vi "run.vi"(8 "error in (no error)":errorcluster, 11 "Filter_Wheel in":refnum<class "Filter_Wheel.lvclass">) -> (0 "error out":errorcluster, 3 "Filter_Wheel out":refnum<class "Filter_Wheel.lvclass">)   [LabVIEW 2018, in "Filter_Wheel.lvclass"]
uses:
  Filter_Wheel.lvclass
  Filter_Wheel.lvclass/Filter_Wheel.ctl
  State Machine/State Machine.lvclass/State Machine.ctl
  State Machine/State Machine.lvclass
  RxTx/RxTx.lvclass
panel:
  out "Select Filter":u16(ring) items=["Methane", "U", "B", "V", "R", "I", "Clear"]
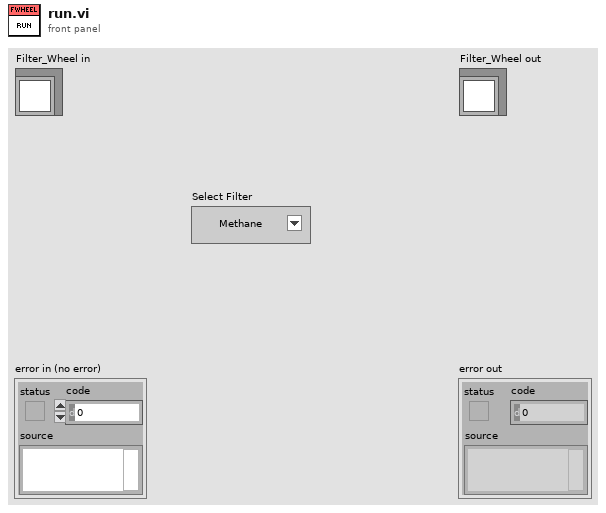
[diagram p1: front panel]
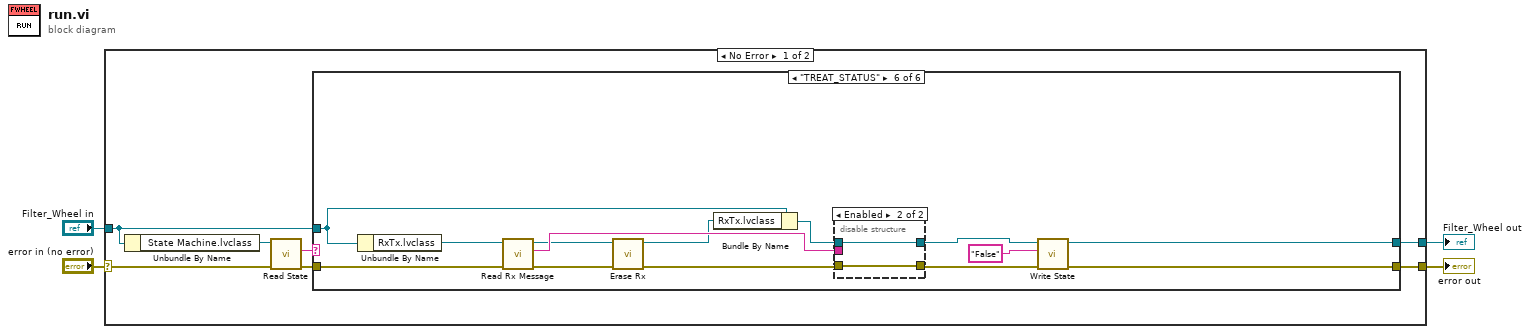
[diagram p0: block diagram]
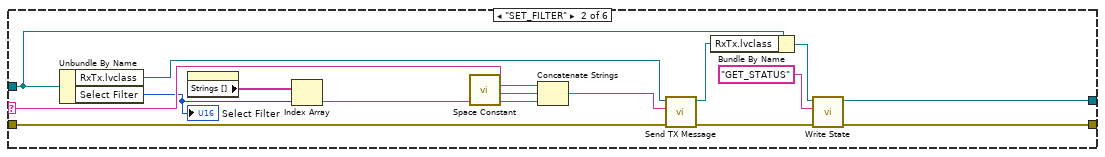
[diagram p3: hidden frame]
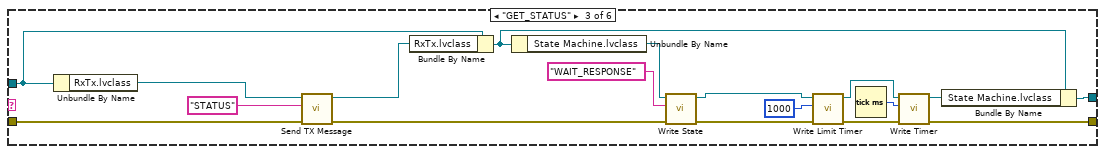
[diagram p4: hidden frame]
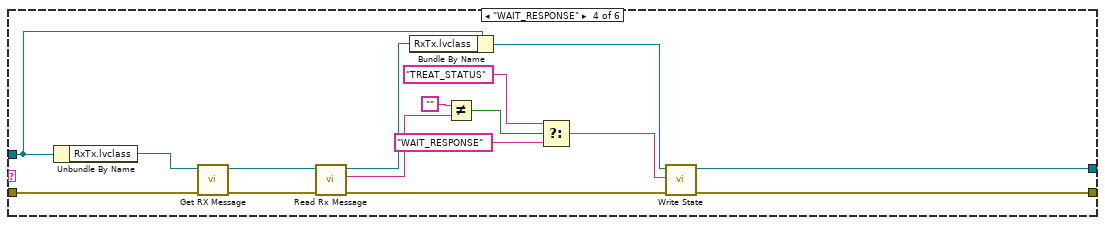
[diagram p5: hidden frame]
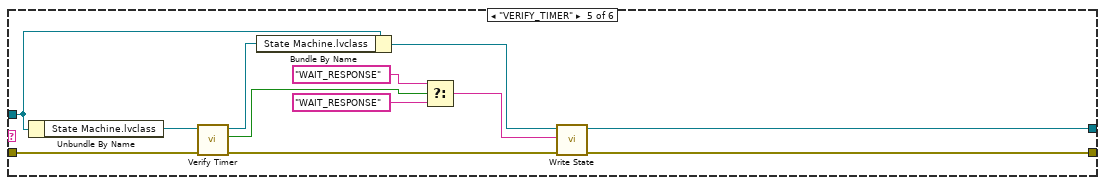
[diagram p6: hidden frame]
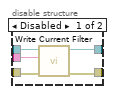
[diagram p7: hidden frame]
diagram:
  n1 = case shown="No Error" "error in (no error)" {
    selector: "error in (no error)" -> [w10 w97]
    tunnel: [w5 w97] -> w3
    tunnel: [w6 w96] -> w1
    tunnel: "Filter_Wheel in" -> [w8 w96]
    frame No Error {
      n2 = Unbundle By Name(w8) -> ("State Machine.lvclass"=w11:refnum<class "State Machine.lvclass">)
      n3 = call-dynamic "Read State.vi"("error in (no error)"=w10, "State Machine in"=w11) -> ("error out"=w7:errorcluster, "State"=w9:string)  [unwired: 7 in, 1 out]
      n4 = case shown="\"TREAT_STATUS\"" w9 {
        selector: w9 -> [_ w27 _ _ _ _]
        tunnel: w8 -> [w13 w24 w42 w62 w74 w88]
        tunnel: w7 -> [w12 w25 w46 w57 w66 w84]
        tunnel: [w13 w18 w37 w59 w71 w86] -> w6
        tunnel: [w12 w19 w38 w60 w72 w87] -> w5
        frame "False", Default {
        }
        frame "SET_FILTER" {
          n5 = Unbundle By Name(w24) -> ("RxTx.lvclass"=w22:refnum<class "RxTx.lvclass">, "Select Filter"=w15:u16)
          "Select Filter" <- w15
          n6 = property on="Select Filter" class="Ring (strict)"() -> ("Strings []"=w16:string[])  [unwired: 2 in, 2 out]
          n7 = Index Array(array=w16, index=w15) -> (element=w14:string)
          n8 = call <vilib>:"Space Constant.vi"() -> ("String"=w26:string)
          n9 = Concatenate Strings(w27, w26, w14) -> (w28:string)
          n10 = call "Send TX Message.vi"("error in (no error)"=w25, "element"=w28, "RxTx in"=w22) -> ("error out"=w20:errorcluster, "RxTx out"=w23:refnum<class "RxTx.lvclass">)  [unwired: 7 in]
          n11 = Bundle By Name(cluster=w24, "RxTx.lvclass"=w23) -> (w21:refnum<class "Filter_Wheel.lvclass">)
          n12 = call "Write State.vi"("error in (no error)"=w20, "State"="GET_STATUS", "Filter_Wheel in"=w21) -> ("error out"=w19:errorcluster, "Filter_Wheel out"=w18:refnum<class "Filter_Wheel.lvclass">)  [unwired: 7 in]
        }
        frame "GET_STATUS" {
          n13 = Unbundle By Name(w42) -> ("RxTx.lvclass"=w44:refnum<class "RxTx.lvclass">)
          n14 = call "Send TX Message.vi"("error in (no error)"=w46, "element"="STATUS", "RxTx in"=w44) -> ("error out"=w41:errorcluster, "RxTx out"=w45:refnum<class "RxTx.lvclass">)  [unwired: 7 in]
          n15 = Bundle By Name(cluster=w42, "RxTx.lvclass"=w45) -> (w32:refnum<class "Filter_Wheel.lvclass">)
          n16 = Unbundle By Name(w32) -> ("State Machine.lvclass"=w33:refnum<class "State Machine.lvclass">)
          n17 = call-dynamic "Write State.vi"("error in (no error)"=w41, "State"="WAIT_RESPONSE", "State Machine in"=w33) -> ("error out"=w40:errorcluster, "State Machine out"=w34:refnum<class "State Machine.lvclass">)  [unwired: 7 in]
          n18 = call "Write Limit Timer.vi"("error in (no error)"=w40, "Limit Timer"=u32 1000, "State Machine in"=w34) -> ("error out"=w39:errorcluster, "State Machine out"=w35:refnum<class "State Machine.lvclass">)  [unwired: 7 in]
          n19 = Tick Count (ms)() -> (millisecond timer value=w29:u32)
          n20 = call "Write Timer.vi"("error in (no error)"=w39, "Timer"=w29, "State Machine in"=w35) -> ("error out"=w38:errorcluster, "State Machine out"=w36:refnum<class "State Machine.lvclass">)  [unwired: 7 in]
          n21 = Bundle By Name(cluster=w32, "State Machine.lvclass"=w36) -> (w37:refnum<class "Filter_Wheel.lvclass">)
        }
        frame "WAIT_RESPONSE" {
          n22 = Unbundle By Name(w62) -> ("RxTx.lvclass"=w58:refnum<class "RxTx.lvclass">)
          n23 = call "Get RX Message.vi"("error in (no error)"=w57, "RxTx in"=w58) -> ("error out"=w56:errorcluster, "RxTx out"=w55:refnum<class "RxTx.lvclass">)  [unwired: 8 in]
          n24 = call "Read Rx Message.vi"("error in (no error)"=w56, "RxTx in"=w55) -> ("error out"=w48:errorcluster, "Rx Message"=w54:string, "RxTx out"=w47:refnum<class "RxTx.lvclass">)  [unwired: 7 in]
          n25 = Bundle By Name(cluster=w62, "RxTx.lvclass"=w47) -> (w61:refnum<class "Filter_Wheel.lvclass">)
          n26 = Not Equal?(x="", y=w54) -> (x != y?=w52:bool)
          n27 = Select(t="TREAT_STATUS" ("State"), s=w52, f="WAIT_RESPONSE" ("State")) -> (s? t:f=w49:string)
          n28 = call "Write State.vi"("error in (no error)"=w48, "State"=w49, "Filter_Wheel in"=w61) -> ("error out"=w60:errorcluster, "Filter_Wheel out"=w59:refnum<class "Filter_Wheel.lvclass">)  [unwired: 7 in]
        }
        frame "VERIFY_TIMER" {
          n29 = Unbundle By Name(w74) -> ("State Machine.lvclass"=w67:refnum<class "State Machine.lvclass">)
          n30 = call "Verify Timer.vi"("error in (no error)"=w66, "State Machine in"=w67) -> ("error out"=w65:errorcluster, "time out"=w63:bool, "State Machine out"=w64:refnum<class "State Machine.lvclass">)  [unwired: 7 in]
          n31 = Bundle By Name(cluster=w74, "State Machine.lvclass"=w64) -> (w73:refnum<class "Filter_Wheel.lvclass">)
          n32 = Select(t="WAIT_RESPONSE" ("State"), s=w63, f="WAIT_RESPONSE" ("State")) -> (s? t:f=w68:string)
          n33 = call "Write State.vi"("error in (no error)"=w65, "State"=w68, "Filter_Wheel in"=w73) -> ("error out"=w72:errorcluster, "Filter_Wheel out"=w71:refnum<class "Filter_Wheel.lvclass">)  [unwired: 7 in]
        }
        frame "TREAT_STATUS" {
          n34 = Unbundle By Name(w88) -> ("RxTx.lvclass"=w85:refnum<class "RxTx.lvclass">)
          n35 = call "Read Rx Message.vi"("error in (no error)"=w84, "RxTx in"=w85) -> ("error out"=w78:errorcluster, "Rx Message"=w79:string, "RxTx out"=w75:refnum<class "RxTx.lvclass">)  [unwired: 7 in]
          n36 = call "Erase Rx.vi"("error in (no error)"=w78, "RxTx in"=w75) -> ("error out"=w77:errorcluster, "RxTx out"=w76:refnum<class "RxTx.lvclass">)  [unwired: 8 in]
          n37 = Bundle By Name(cluster=w88, "RxTx.lvclass"=w76) -> (w80:refnum<class "Filter_Wheel.lvclass">)
          n38 = disable-structure shown="Enabled" {
            disable-tunnel: [w93 w95] -> w82
            disable-tunnel: [w92 w94] -> w81
            disable-tunnel: w80 -> [w91 w95]
            disable-tunnel: w79 -> [w90 _]
            disable-tunnel: w77 -> [w89 w94]
            frame Disabled {
              n39 = call "Write Current Filter.vi"("error in (no error)"=w89, "Current Filter"=w90, "Filter_Wheel in"=w91) -> ("error out"=w92:errorcluster, "Filter_Wheel out"=w93:refnum<class "Filter_Wheel.lvclass">)  [unwired: 7 in]
            }
            frame Enabled {
            }
          }
          n40 = call "Write State.vi"("error in (no error)"=w81, "State"="False", "Filter_Wheel in"=w82) -> ("error out"=w87:errorcluster, "Filter_Wheel out"=w86:refnum<class "Filter_Wheel.lvclass">)  [unwired: 7 in]
        }
      }
    }
    frame Error {
    }
  }
  "error out" <- w3
  "Filter_Wheel out" <- w1
